vi "_CFX_Sole备份.vi"(0 "CFX cmd":T6, 1 "CFX State":T7, 5 "CFX-config":T2={"neme"="上板机", "CFX Handle"="Cleaner", "Request IP"="amqp://192.168.1.10:5672", "User"="admin", "password"="123456", "Broker IP"="192.168.1.20", "Broker Port"="5672", "Publish Path"="/exchange/Cleaner", "SubPubish Path"="/queue/Broadcast-Cleaner", "Broadcast \nPublish Path"="/exchange/CFX.Host", "Broadcast Sub\npublish Path"="/queue/Broadcast-CFX.Host", "Target \nHandle lD"="CFX.Host", "target IP"="amqp://127.0.0.1", "unit verification"=TRUE, "heartbeat"=FALSE, "timeout period"=5.0}, 7 "CfxData":T1={"Vendor"="YXD", "UniqueIdentifier"="UID5620001", "FriendlyName"="SBJ", "ModelNumber"="SBJ_0001", "SerialNumber"="563210", "NumberofLanes"="2", "CodeIn"="", "CodeOut"="", "Unitldentifer"="", "PositionNumber"="", "PositionName"="", "OldState"="", "NewState"="", "OldStateDuration"="", "Faultcode"="", "Operatorldentifer"="", "LoginName"="", "RecipeName"="", "Revision"="", "Activate formula"="", "Description"=""}, 11 "Error In":errorcluster caption="错误输入", 12 "send?":bool) -> (6 "MessageCFX_out":string, 8 "CFX_Message_In":T3, 14 "ok?":bool, 15 "Error Out":errorcluster caption="错误输出")   [LabVIEW 2025]
uses:
  CFX_dll/CFX.dll
  ctl/CFX-cmd.ctl
  ctl/CfxTopic-cmd.ctl
  ctl/CFX_data.ctl
  ctl/CFX-config.ctl
  SubVI/table/1 model/a log/_myType runlog cmd.ctl
panel:
  out "QueueName":string
  out "IsOpen":bool
  in  "CFX.Host?":bool
  in  "enable?":bool
  out "TraceMessage_EVE":refnum<k27>
  out "TraceMessage":string
  out "AooLog":refnum<k24>
  out "TestSubscribeChannel":bool
  out "TestPublishChannel":bool
  out "log":string
  out "error out":errorcluster
  out "objAMQP_MSG":refnum<k27>
  out "Connection":T4 {"ConnectionEstablished" items=["ConnectionEstablished", "ConnectionFailed", "ConnectionInterrupted", "ConnectionClosed"]}
  out "objAMQP_Request":refnum<k27>
  out "SubscribeChannel":refnum<k24>
  out "return":T5={"CFXHandle"="Cleaner", "RequestNetworkUri"="amqp://10.33.191.97:5672", "RequestTargetAddress"="/queue/Cleaner", "CFX_Message_In"={"Message_Name"="", "Message_Content"=""}, "CFX_Message_out"={"Message_Name"="", "Message_Content"=""}, "CFX_data"=refnum}
  out "FromListener":string
  in  "EndpointInformation":string
  in  "NewState":i32(ring)=1000 items=["PRD"=1000, "PRD_RegularWork"=1100, "PRD_WorkForThirdParties"=1200, "PRD_Rework"=1300, "PRD_Engineering"=1400, "SBY"=2000, "SBY_NoOperator"=2100, "SBY_NoProduct"=2200, "SBY_NoSupportTool"=2300, "SBY_AssociatedClusterModuleDown"=2400, "SBY_NoHost"=2500, "ENG"=3000, "ENG_ProcessExperiments"=3100, "ENG_EquipmentExperiments"=3200, "SDT"=4000, "SDT_UserMaintenanceDelay"=4100, "SDT_SuppliedMaintenanceDelay"=4200, "SDT_PreventiveMaintenance"=4300, "SDT_ChangeOfConsumables"=4400, "SDT_Setup"=4500, "SDT_ProductionTest"=4600, "SDT_FacilitiesRelated"=4700, "USD"=5000, "USD_UserMaintentanceDelay"=5100, "USD_SuppliedMaintenanceDelay"=5200, "USD_Repair"=5300, "USD_OutOfSpecInputMaterial"=5400, "USD_ChangeOfConsumables"=5500, "USD_FacilitiesRelated"=5600, "NST"=6000, "NST_UnworkedShifts"=6100, "NST_EquipmentInstallation"=6200, "NST_EquipmentModifications"=6300, "NST_OfflineTraining"=6400, "NST_ShutdownAndStartup"=6500]
  in  "Broker Url":string="amqp://admin:123456@10.33.191.54:5672"
  out "PublishChannel":refnum<k24>
  in  "rngNewState":i32(ring) items=["PRD"=1000, "PRD_RegularWork"=1100, "PRD_WorkForThirdParties"=1200, "PRD_Rework"=1300, "PRD_Engineering"=1400, "SBY"=2000, "SBY_NoOperator"=2100, "SBY_NoProduct"=2200, "SBY_NoSupportTool"=2300, "SBY_AssociatedClusterModuleDown"=2400, "SBY_NoHost"=2500, "ENG"=3000, "ENG_ProcessExperiments"=3100, "ENG_EquipmentExperiments"=3200, "SDT"=4000, "SDT_UserMaintenanceDelay"=4100, "SDT_SuppliedMaintenanceDelay"=4200, "SDT_PreventiveMaintenance"=4300, "SDT_ChangeOfConsumables"=4400, "SDT_Setup"=4500, "SDT_ProductionTest"=4600, "SDT_FacilitiesRelated"=4700, "USD"=5000, "USD_UserMaintentanceDelay"=5100, "USD_SuppliedMaintenanceDelay"=5200, "USD_Repair"=5300, "USD_OutOfSpecInputMaterial"=5400, "USD_ChangeOfConsumables"=5500, "USD_FacilitiesRelated"=5600, "NST"=6000, "NST_UnworkedShifts"=6100, "NST_EquipmentInstallation"=6200, "NST_EquipmentModifications"=6300, "NST_OfflineTraining"=6400, "NST_ShutdownAndStartup"=6500]
  # "此端点的唯一 CFX 句柄。"
  # "节点队列名"
  # "amqp://10.33.191.64:5672"
  # "amqp://localhost:5672"
  # "Laser"
  # "amqp://192.168.1.20:5672"
  # "AMQP 源或目标的网络地址。可以包括 user 和 port 信息 标准 Uri 格式。（例如：amqps://user1:password1@myamqpbroker.company1.com、amqp://broker3.company1.com、 amqps://myamqpbroker.company1.com:8856 等）。"
  # "本地消息源\nRequest Source"
  # "代理层\nBroker"
  # "请求目标\nRequest Target"
  # "可配置项"
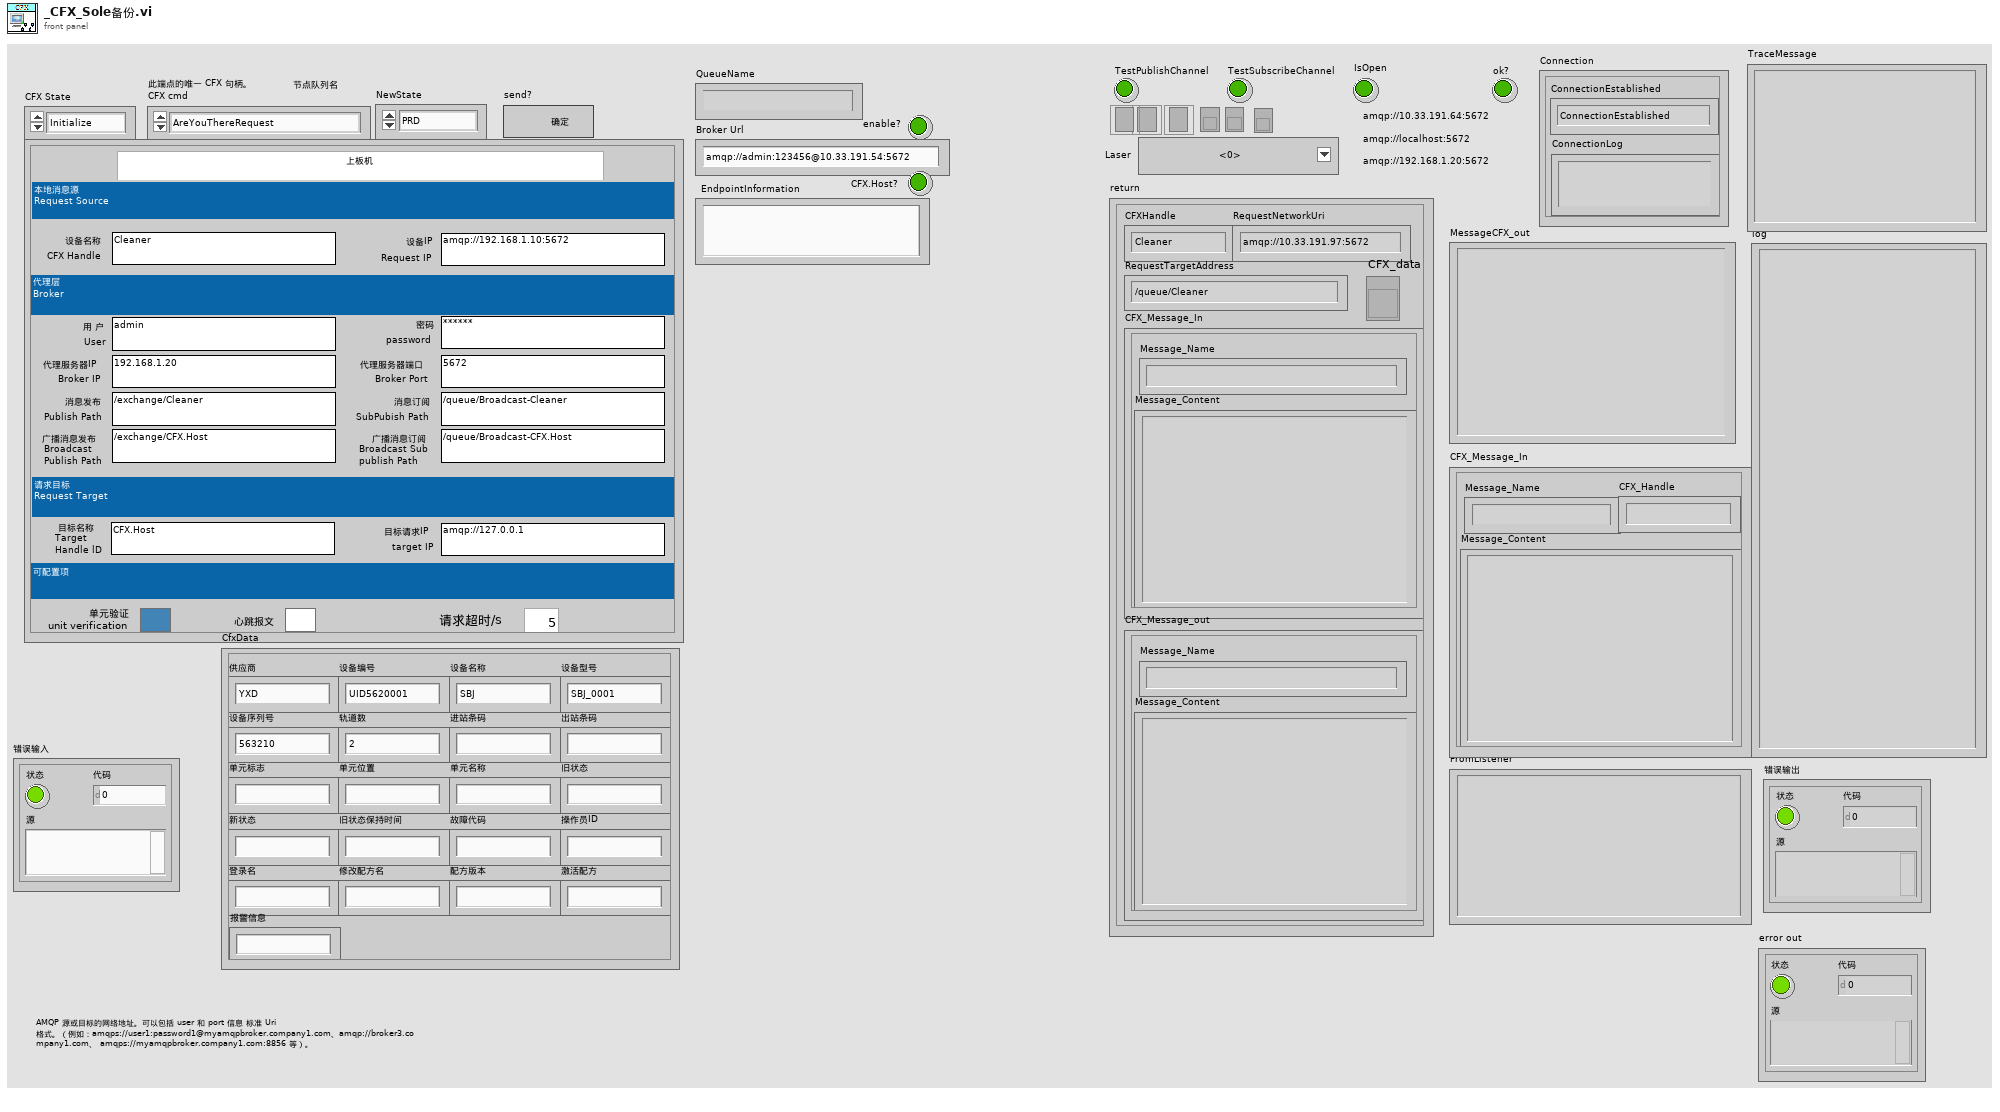
[diagram p1: front panel]
types:
  T1 = typedef "CFX_data.ctl" = cluster{"Vendor":string, "UniqueIdentifier":string, "FriendlyName":string, "ModelNumber":string, "SerialNumber":string, "NumberofLanes":string, "CodeIn":string, "CodeOut":string, "Unitldentifer":string, "PositionNumber":string, "PositionName":string, "OldState":string, "NewState":string, "OldStateDuration":string, "Faultcode":string, "Operatorldentifer":string, "LoginName":string, "RecipeName":string, "Revision":string, "Activate formula":string, "Description":string}
  T2 = typedef "CFX-config.ctl" = cluster{"neme":string, "CFX Handle":string, "Request IP":string, "User":string, "password":string, "Broker IP":string, "Broker Port":string, "Publish Path":string, "SubPubish Path":string, "Broadcast \nPublish Path":string, "Broadcast Sub\npublish Path":string, "Target \nHandle lD":string, "target IP":string, "unit verification":bool, "heartbeat":bool, "timeout period":dbl}
  T3 = cluster{"Message_Name":string, "CFX_Handle":string, "Message_Content":string}
  T4 = cluster{"ConnectionEstablished":i32, "ConnectionLog":string}
  T5 = cluster{"CFXHandle":string, "RequestNetworkUri":string, "RequestTargetAddress":string, "CFX_Message_In":cluster{"Message_Name":string, "Message_Content":string}, "CFX_Message_out":cluster{"Message_Name":string, "Message_Content":string}, "CFX_data":refnum<vi>}
  T6 = typedef "CfxTopic-cmd.ctl" = enum16{"AreYouThereRequest", "AreYouThereResponse", "EndpointConnected", "EndpointShuttingDown", "GetEndpointInformationRequest", "GetEndpointInformationResponse", "Heartbeat", "NotSupportedResponse", "WhoIsThereRequest", "WhoIsThereResponse", "UnitArrived", "UnitsDeparted", "StationStateChanged", "FaultOccurred", "FaultCleared", "OperatorActivated", "OperatorDeactivated", "RecipeModified", "RecipeActived", "ActivateRecipeRequest", "ActivateRecipeResponse"}
  T7 = typedef "CFX-cmd.ctl" = enum16{"Initialize", "Event", "Connection test", "OpenConnection", "Idle", "Shutdown", "WorkComplete", "StationStateChanged", "MaterialsApplied", "CFX", "Hermes"}
  T8 = typedef "_myType runlog cmd.ctl" = enum16{"init", "push (-1: error)", "push (0: user)", "push (1: logical)", "push (2: driver)", "push (3: lib-core)", "push (4: reserved)", "pop", "more?"}
  T9 = cluster{"CFXHandle":string, "RequestNetworkUri":string, "RequestTargetAddress":string, "CFX_Message_In":cluster{"Message_Name":string, "Message_Content":string}, "CFX_Message_out":cluster{"Message_Name":string, "Message_Content":string}, "CFX_data 2":refnum<vi>}
  T10 = typedef "LVStringsAndValuesArrayTypeDef_I32.ctl" = cluster{"String":string, "Value":i32}[]
  T11 = cluster{"Message_Name":string, "Message_Content":string}
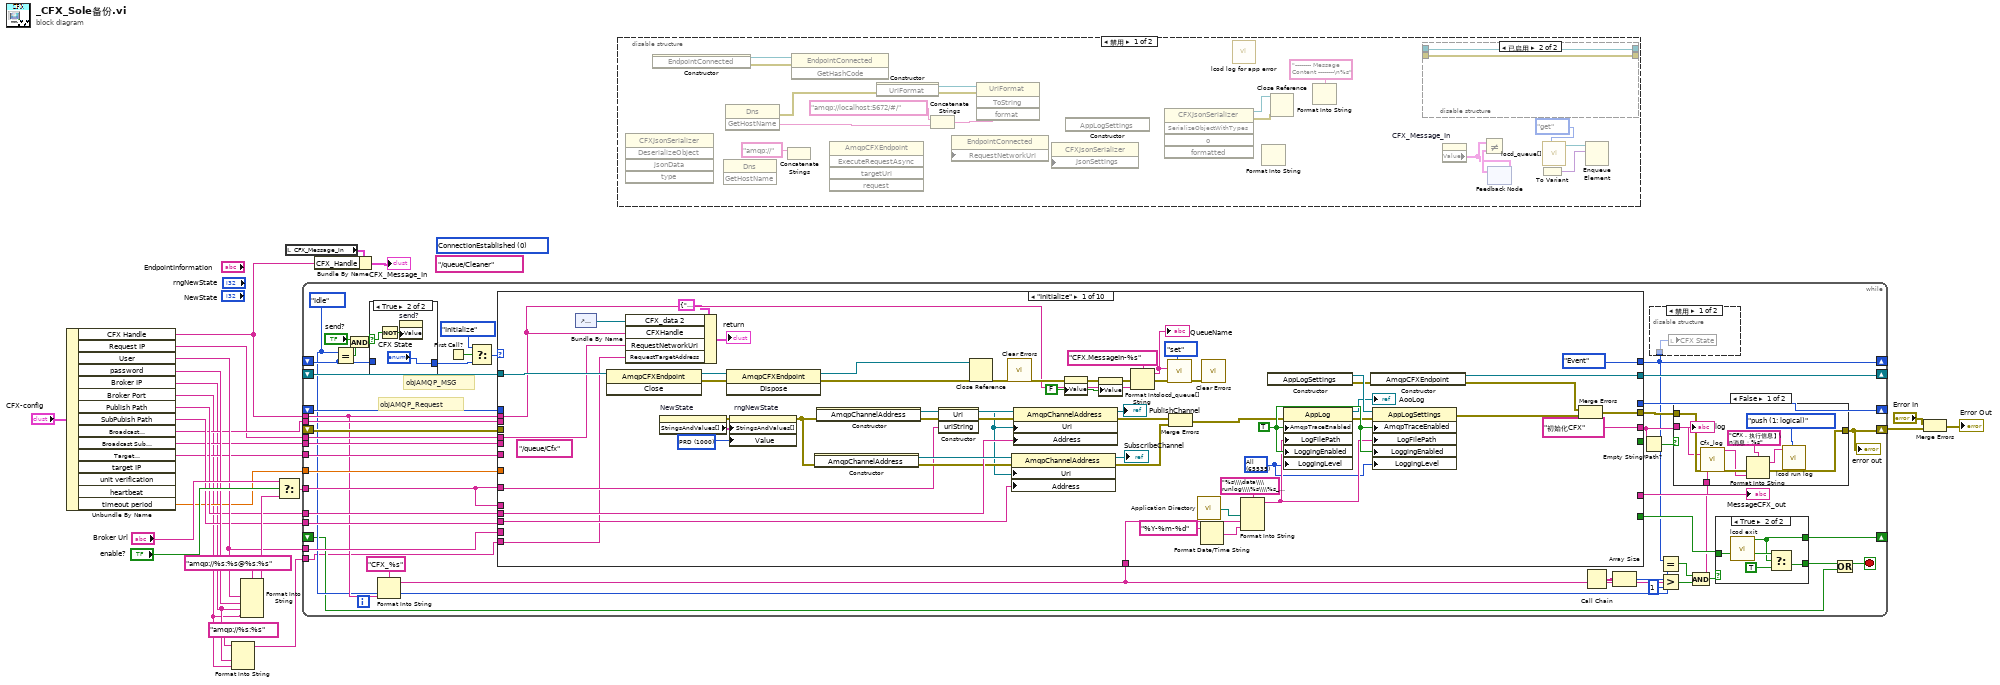
[diagram p0: block diagram]
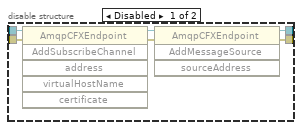
[diagram p2: hidden frame]
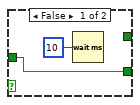
[diagram p6: hidden frame]
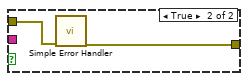
[diagram p7: hidden frame]
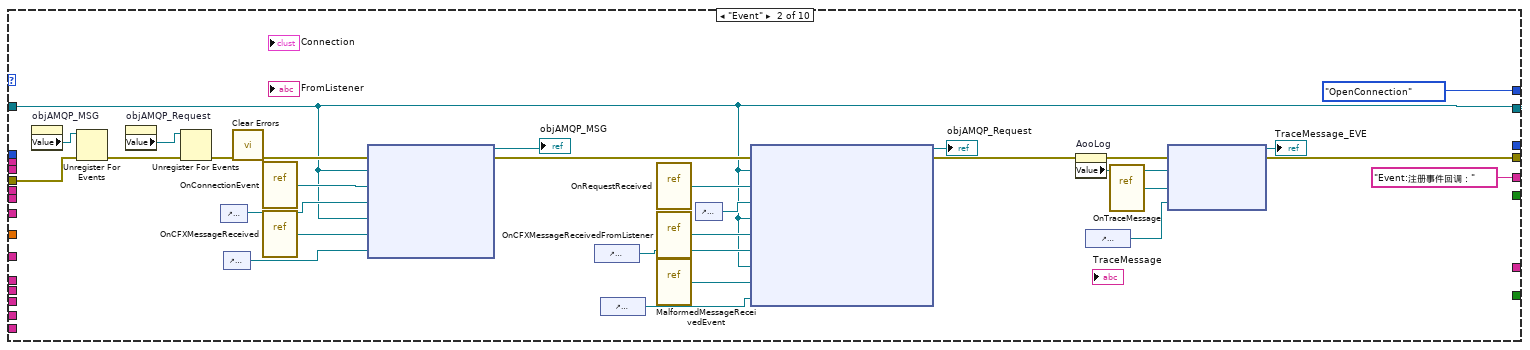
[diagram p8: hidden frame]
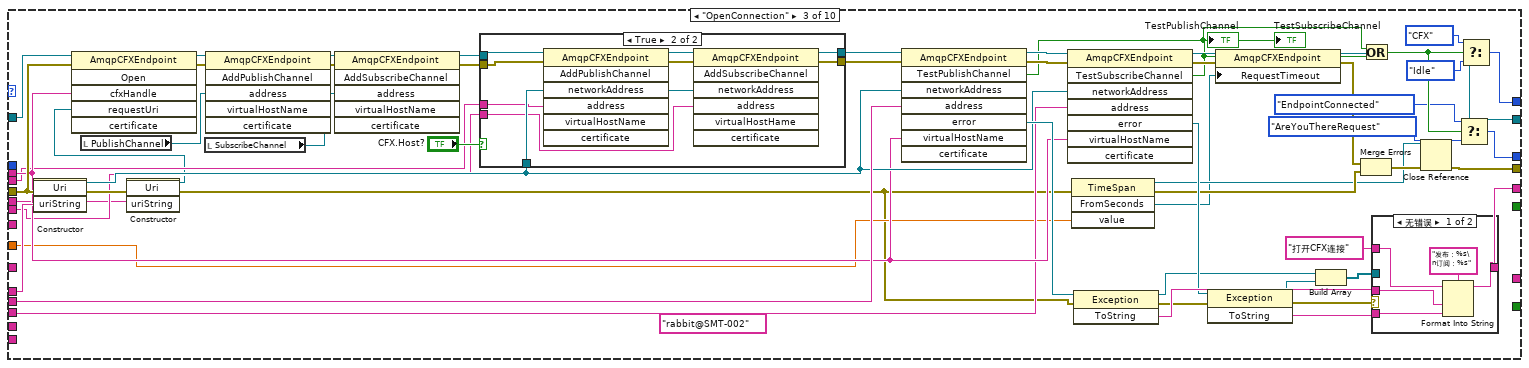
[diagram p9: hidden frame]
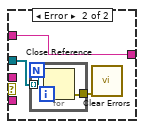
[diagram p11: hidden frame]
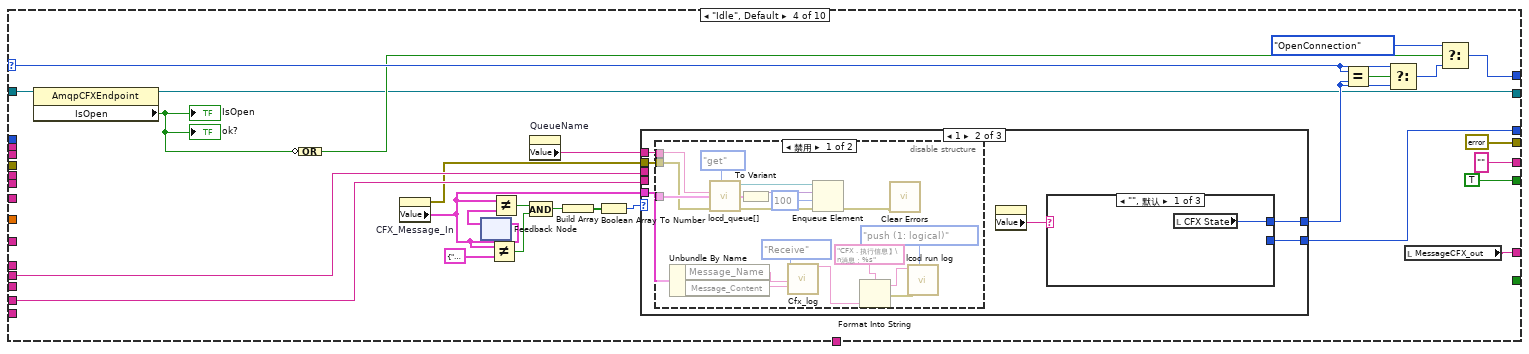
[diagram p12: hidden frame]
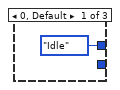
[diagram p13: hidden frame]
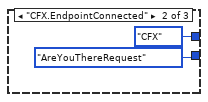
[diagram p15: hidden frame]
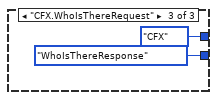
[diagram p16: hidden frame]
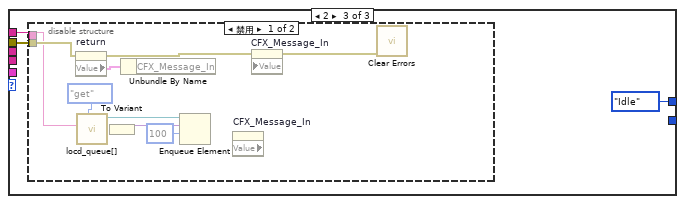
[diagram p17: hidden frame]
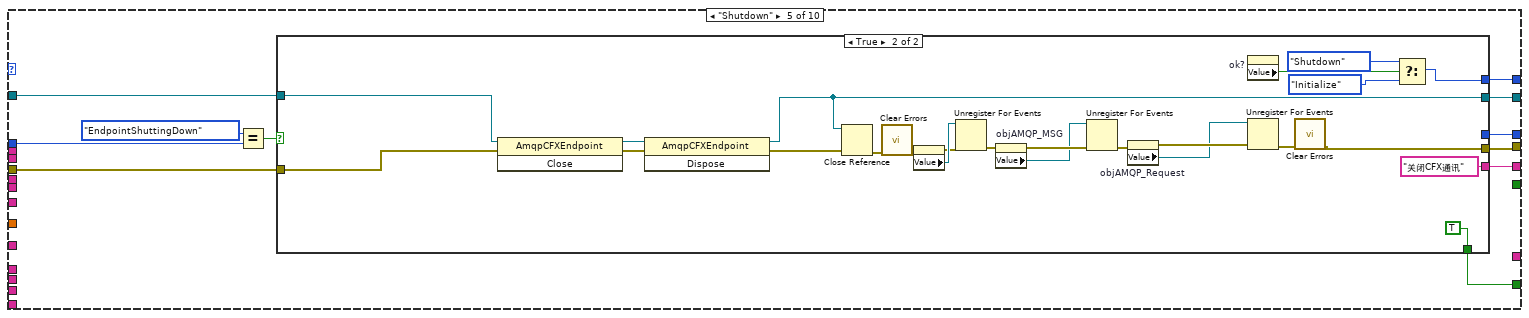
[diagram p19: hidden frame]
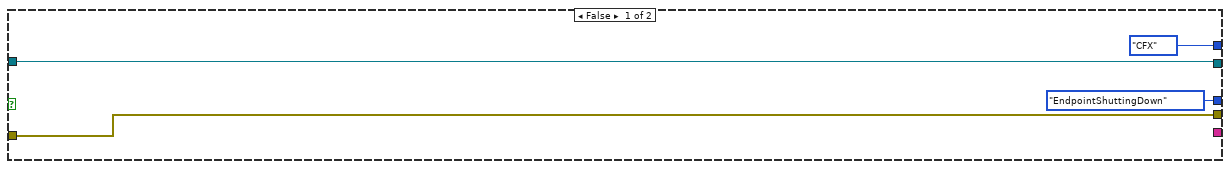
[diagram p20: hidden frame]
diagram:
  (unwired) "/queue/Cleaner" ("RequestTargetAddress")
  (unwired) 0 items=["ConnectionEstablished", "ConnectionFailed", "ConnectionInterrupted", "ConnectionClosed"] ("ConnectionEstablished")
  n1 = Unbundle By Name("CFX-config") -> ("CFX Handle"=w7:string, "Request IP"=w10:string, "User"=w18:string, "password"=w17:string, "Broker IP"=w3:string, "Broker Port"=w2:string, "Publish Path"=w16:string, "SubPubish Path"=w15:string, "Broadcast \nPublish Path"=w14:string, "Broadcast Sub\npublish Path"=w13:string, "Target \nHandle lD"=w12:string, "timeout period"=w11:dbl)  [unwired: 3 out]
  n2 = Format Into String(format string="amqp://%s:%s" ("格式字符串"), w3, w2) -> (resulting string=w1:string)  [unwired: 2 in, 1 out]
  n3 = Format Into String(format string="amqp://%s:%s@%s:%s" ("格式字符串"), w18, w17, w3, w2) -> (resulting string=w20:string)  [unwired: 2 in, 1 out]
  n4 = Select(t="Broker Url", s="enable?", f=w20) -> (s? t:f=w9:string)
  n5 = local read "CFX_Message_In"() -> (w6:T3)
  n6 = while {
    shift-right: [w45] -> _
    shift-left: _ -> [w34]
    shift-right: [w68] -> _
    shift-left: _ -> [w69]
    shift-right: [w62] -> w8
    shift-left: _ -> [w56]
    shift-right: [w61] -> _
    shift-left: _ -> [w63]
    tunnel: w9 -> [w57]
    tunnel: w15 -> [w60]
    tunnel: w16 -> [w59]
    tunnel: w7 -> [w39]
    tunnel: w18 -> [w58]
    tunnel: w10 -> [w55]
    tunnel: w14 -> [w54]
    tunnel: w13 -> [w53]
    tunnel: w12 -> [w52]
    tunnel: w11 -> [w51]
    shift-right: [w35] -> _
    shift-left: _ -> [w29]
    tunnel: w1 -> [w26]
    stop <- w30 stop-if-true
    w33 = CFX-cmd."Idle" ("CFX State")
    # "objAMQP_Request"
    # "objAMQP_MSG"
    n7 = Equal?(x=w33, y=w34) -> (x = y?=w31:bool)
    n8 = And(x="send?", y=w31) -> (x .and. y?=w32:bool)
    n9 = case shown="True" w32 {
      selector: w32 -> [_ w73]
      tunnel: w34 -> [w71 _]
      tunnel: [w71 "CFX State"] -> w38
      frame False {
      }
      frame True {
        n10 = Not(x=w73) -> (.not. x?=w72:bool)
        n11 = property on="send?" class="Bool (严格)"("Value"=w72) -> ()  [unwired: 2 in, 2 out]
      }
    }
    n12 = Format Into String(format string="CFX_%s" ("log_path"), w39) -> (resulting string=w37:string)  [unwired: 2 in, 1 out]
    n13 = First Call?() -> (First Call?: T/F=w27:bool)
    n14 = Select(t=CFX-cmd."Initialize" ("CFX State"), s=w27, f=w38) -> (s? t:f=w41:T7)
    n15 = case shown="\"Initialize\"" w41 {
      selector: w41 -> [_ _ _ w280 _ _ _ _ _ _]
      tunnel: [_ _ _ _ w326 _ _ _ _ _] -> w47
      tunnel: w69 -> [w128 w149 w232 w269 w332 w376 w404 w429 w469 w487]
      tunnel: [w134 w149 w189 w254 w328 w375 w402 w428 w468 w486] -> w68
      tunnel: [w129 w168 w203 errorcluster {"status"=FALSE, "code"=0, "source"=""} ("error out") w327 w372 w399 w427 w479 w485] -> w67
      tunnel: [_ _ _ w279 _ w367 w391 w414 w463 w484] -> w66
      tunnel: [_ _ _ TRUE _ _ _ _ _ _] -> _
      tunnel: ["初始化CFX" ("格式字符串") "Event:注册事件回调：" ("SerializeObjectWithTypes") w225 "" ("SerializeObjectWithTypes") w331 w364 w391 w413 w473 w484] -> w65
      tunnel: [CFX-cmd."Event" ("CFX State") CFX-cmd."OpenConnection" ("CFX State") w196 w264 w330 CFX-cmd."Idle" ("CFX State") CFX-cmd."Idle" ("CFX State") CFX-cmd."Idle" ("CFX State") w449 CFX-cmd."Idle" ("CFX State")] -> w45
      tunnel: w56 -> [_ w163 w206 _ w329 w362 w389 w411 w470 w482]
      tunnel: w63 -> [_ _ _ _ w325 _ _ _ w453 _]
      tunnel: [_ _ w192 w274 w322 _ _ _ w448 _] -> w61
      tunnel: w57 -> [w101 _ _ _ _ _ _ _ _ _]
      tunnel: w60 -> [w119 _ w185 _ _ _ _ _ _ _]
      tunnel: w59 -> [w118 _ w215 w271 _ _ _ _ _ _]
      tunnel: w39 -> [w104 _ w199 _ _ _ _ _ w446 _]
      tunnel: w58 -> [_ _ _ w270 _ _ _ _ _ _]
      tunnel: w57 -> [_ _ w214 _ _ _ _ _ _ _]
      tunnel: w55 -> [w105 _ w183 _ _ _ _ _ _ _]
      tunnel: w54 -> [_ _ w187 _ _ _ _ _ _ _]
      tunnel: w53 -> [_ _ w186 _ _ _ _ _ _ _]
      tunnel: w52 -> [_ _ _ _ _ _ _ _ w445 _]
      tunnel: w51 -> [_ _ w184 _ _ _ _ _ _ _]
      tunnel: w37 -> [w103 _ _ _ _ _ _ _ _ _]
      tunnel: w26 -> [w94 _ _ _ _ _ _ _ _ _]
      frame "Initialize" {
        (unwired) "/queue/Cfx" ("RequestTargetAddress")
        w123 = FALSE ("TestPublishChannel")
        w131 = 65535 items=["Debug"=1, "Info"=2, "Warn"=4, "Error"=8, "All"=65535] ("LoggingLevel")
        w133 = TRUE ("LoggingEnabled")
        w145 = 1000 items=["PRD"=1000, "PRD_RegularWork"=1100, "PRD_WorkForThirdParties"=1200, "PRD_Rework"=1300, "PRD_Engineering"=1400, "SBY"=2000, "SBY_NoOperator"=2100, "SBY_NoProduct"=2200, "SBY_NoSupportTool"=2300, "SBY_AssociatedClusterModuleDown"=2400, "SBY_NoHost"=2500, "ENG"=3000, "ENG_ProcessExperiments"=3100, "ENG_EquipmentExperiments"=3200, "SDT"=4000, "SDT_UserMaintenanceDelay"=4100, "SDT_SuppliedMaintenanceDelay"=4200, "SDT_PreventiveMaintenance"=4300, "SDT_ChangeOfConsumables"=4400, "SDT_Setup"=4500, "SDT_ProductionTest"=4600, "SDT_FacilitiesRelated"=4700, "USD"=5000, "USD_UserMaintentanceDelay"=5100, "USD_SuppliedMaintenanceDelay"=5200, "USD_Repair"=5300, "USD_OutOfSpecInputMaterial"=5400, "USD_ChangeOfConsumables"=5500, "USD_FacilitiesRelated"=5600, "NST"=6000, "NST_UnworkedShifts"=6100, "NST_EquipmentInstallation"=6200, "NST_EquipmentModifications"=6300, "NST_OfflineTraining"=6400, "NST_ShutdownAndStartup"=6500] ("NewState")
        n16 = control-ref of="CfxData"() -> (w93:refnum<vi>)
        n17 = invoke class="AmqpCFXEndpoint" method="Close"(reference=w128) -> (reference out=w126:refnum<k24>, error out=w95:errorcluster)  [unwired: 2 in, 1 out]
        n18 = Bundle By Name(cluster=T9 {"CFXHandle"="Cleaner", "RequestNetworkUri"="amqp://192.168.1.10:5672", "RequestTargetAddress"="/queue/Cleaner", "CFX_Message_In"={"Message_Name"="", "Message_Content"=""}, "CFX_Message_out"={"Message_Name"="", "Message_Content"=""}, "CFX_data 2"=refnum} ("return"), "CFX_data 2"=w93, "CFXHandle"=w104, "RequestNetworkUri"=w105, "RequestTargetAddress"=w94) -> (→"return":T9)
        n19 = property on="NewState" class="Ring (严格)"() -> (error out=w144:errorcluster, "StringsAndValues[]"=w148:T10)  [unwired: 2 in, 1 out]
        n20 = invoke on="调用节点" class="AmqpCFXEndpoint" method="Dispose"(reference=w126, error in=w95) -> (reference out=w97:refnum<k24>, error out=w96:errorcluster)  [unwired: 1 in, 1 out]
        n21 = property on="rngNewState" class="Ring (严格)"(error in=w144, "StringsAndValues[]"=w148, "Value"=w145) -> (error out=w125:errorcluster)  [unwired: 1 in, 1 out]
        n22 = constructor class="AmqpChannelAddress"(error in=w125) -> (reference out=w138:refnum<k24>, error out=w117:errorcluster)  [unwired: 2 in, 1 out]
        n23 = constructor class="AmqpChannelAddress"(error in=w125) -> (reference out=w143:refnum<k24>, error out=w147:errorcluster)  [unwired: 2 in, 1 out]
        n24 = constructor class="Uri"(error in=w147, "uriString"=w101) -> (reference out=w116:refnum<k24>, error out=w146:errorcluster)  [unwired: 2 in, 2 out]
        n25 = Close Reference(reference=w97, error in (no error)=w96) -> (error out=w127:errorcluster)
        n26 = call <vilib>:"Clear Errors.vi"("error in (no error)"=w127) -> ("error out"=w115:errorcluster)  [unwired: 5 in, 1 out]
        n27 = property class="AmqpChannelAddress"(reference=w138, error in=w117, "Uri"=w116, "Address"=w119) -> (reference out=→"SubscribeChannel":refnum<k24>, error out=w136:errorcluster)
        n28 = property class="AmqpChannelAddress"(reference=w143, error in=w146, "Uri"=w116, "Address"=w118) -> (reference out=→"PublishChannel":refnum<k24>, error out=w137:errorcluster)
        n29 = property on="TestPublishChannel" class="Bool (严格)"(error in=w115, "Value"=w123) -> (error out=w124:errorcluster)  [unwired: 1 in, 1 out]
        n30 = property on="TestSubscribeChannel" class="Bool (严格)"(error in=w124, "Value"=w123) -> (error out=w100:errorcluster)  [unwired: 1 in, 1 out]
        n31 = Format Into String(format string="CFX.MessageIn-%s" ("格式字符串"), error in=w100, w104) -> (resulting string=w109:string, error out=w106:errorcluster)  [unwired: 1 in]
        "QueueName" <- w109
        n32 = call "locd_queue[].vi"("cmd"=enum16{"init", "get", "set", "end"}."set", "error in"=w106, "queue_name"=w109) -> ("error out"=w107:errorcluster)  [unwired: 4 in, 4 out]
        n33 = Merge Errors(w137, w136) -> (w108:errorcluster)
        n34 = call <vilib>:"Application Directory.vi"() -> ("Application Directory"=w142:path)
        n35 = Format Date/Time String(time format string (%c)="%Y-%m-%d" ("格式字符串")) -> (date/time string=w102:string)  [unwired: 2 in]
        n36 = call <vilib>:"Clear Errors.vi"("error in (no error)"=w107) -> ()  [unwired: 5 in, 2 out]
        n37 = Format Into String(format string="%s\\\\data\\\\runlog\\\\%s\\\\%s_cfxDebig.txt" ("格式字符串"), w142, w103, w102) -> (resulting string=w132:string)  [unwired: 2 in, 1 out]
        n38 = constructor class="AppLogSettings"() -> (reference out=w130:refnum<k24>, error out=w122:errorcluster)  [unwired: 3 in, 1 out]
        n39 = property class="AppLog"(error in=w108, "AmqpTraceEnabled"=w133, "LogFilePath"=w132, "LoggingEnabled"=w133, "LoggingLevel"=w131) -> (reference out=→"AooLog":refnum<k24>, error out=w120:errorcluster)  [unwired: 1 in]
        n40 = constructor class="AmqpCFXEndpoint"(error in=w122) -> (reference out=w134:refnum<k24>, error out=w98:errorcluster)  [unwired: 2 in, 1 out]
        n41 = property class="AppLogSettings"(reference=w130, error in=w120, "AmqpTraceEnabled"=w133, "LogFilePath"=w132, "LoggingEnabled"=w133, "LoggingLevel"=w131) -> (error out=w112:errorcluster)  [unwired: 1 out]
        n42 = Merge Errors(w98, w112) -> (w129:errorcluster)
      }
      frame "Event" {
        n43 = property on="objAMQP_MSG" class="Ref (严格)"() -> ("Value"=w152:refnum<k27>)  [unwired: 2 in, 2 out]
        n44 = Unregister For Events(event registration refnum=w152, error in=w163) -> (error out=w153:errorcluster)
        n45 = property on="objAMQP_Request" class="Ref (严格)"() -> ("Value"=w150:refnum<k27>)  [unwired: 2 in, 2 out]
        n46 = Unregister For Events(event registration refnum=w150, error in=w153) -> (error out=w151:errorcluster)
        n47 = control-ref of="Connection"() -> (w175:refnum<vi>)
        n48 = control-ref of="CFX_Message_In"() -> (w160:refnum<vi>)
        n49 = call <vilib>:"Clear Errors.vi"("error in (no error)"=w151) -> ("error out"=w154:errorcluster)  [unwired: 5 in, 1 out]
        n50 = vi-ref "OnConnectionEvent.vi"() -> ("vi reference"=w176:refnum<vi>)
        n51 = vi-ref "OnCFXMessageReceived.vi"() -> ("vi reference"=w161:refnum<vi>)
        n52 = node(w154, w149, w176, w175, w149, w161, w160) -> (→"objAMQP_MSG":refnum<k27>, w159:errorcluster)  [unwired: 1 in]
        n53 = control-ref of="FromListener"() -> (w157:refnum<vi>)
        n54 = control-ref of="FromListener"() -> (w155:refnum<vi>)
        n55 = vi-ref "OnRequestReceived.vi"() -> ("vi reference"=w174:refnum<vi>)
        n56 = vi-ref "OnCFXMessageReceivedFromListener.vi"() -> ("vi reference"=w158:refnum<vi>)
        n57 = vi-ref "MalformedMessageReceivedEvent.vi"() -> ("vi reference"=w156:refnum<vi>)
        n58 = control-ref of="return"() -> (w165:refnum<vi>)
        n59 = node(w159, w149, w174, w165, w149, w158, w157, w149, w156, w155) -> (→"objAMQP_Request":refnum<k27>, w162:errorcluster)  [unwired: 1 in]
        n60 = property on="AooLog" class="Ref (严格)"(error in=w162) -> (error out=w164:errorcluster, "Value"=w170:refnum<k24>)  [unwired: 1 in, 1 out]
        n61 = control-ref of="TraceMessage"() -> (w166:refnum<vi>)
        n62 = vi-ref "OnTraceMessage.vi"() -> ("vi reference"=w169:refnum<vi>)
        n63 = node(w164, w170, w169, w166) -> (→"TraceMessage_EVE":refnum<k27>, w168:errorcluster)  [unwired: 1 in]
      }
      frame "OpenConnection" {
        (unwired) "rabbit@SMT-002" ("sourceAddress")
        n64 = constructor class="Uri"(error in=w206, "uriString"=w214) -> (reference out=w213:refnum<k24>, error out=w211:errorcluster)  [unwired: 2 in, 2 out]
        n65 = local read "PublishChannel"() -> (w227:refnum<k24>)
        n66 = constructor class="Uri"(error in=w211, "uriString"=w183) -> (reference out=w179:refnum<k24>, error out=w178:errorcluster)  [unwired: 2 in, 2 out]
        n67 = invoke class="AmqpCFXEndpoint" method="Open"(reference=w232, error in=w206, "cfxHandle"=w199, "requestUri"=w179) -> (reference out=w210:refnum<k24>, error out=w209:errorcluster)  [unwired: 2 in, 4 out]
        n68 = local read "SubscribeChannel"() -> (w228:refnum<k24>)
        n69 = invoke class="AmqpCFXEndpoint" method="AddPublishChannel"(reference=w210, error in=w209, "address"=w227) -> (reference out=w231:refnum<k24>, error out=w230:errorcluster)  [unwired: 3 in, 4 out]
        n70 = invoke class="AmqpCFXEndpoint" method="AddSubscribeChannel"(reference=w231, error in=w230, "address"=w228) -> (reference out=w207:refnum<k24>, error out=w200:errorcluster)  [unwired: 3 in, 4 out]
        n71 = case shown="True" "CFX.Host?" {
          tunnel: w213 -> [_ w243]
          tunnel: [w233 w242] -> w212
          tunnel: [w234 w241] -> w208
          tunnel: w207 -> [w234 w240]
          tunnel: w200 -> [w233 w237]
          tunnel: w187 -> [_ w236]
          tunnel: w186 -> [_ w235]
          frame False {
          }
          frame True {
            n72 = invoke class="AmqpCFXEndpoint" method="AddPublishChannel"(reference=w240, error in=w237, "networkAddress"=w243, "address"=w236) -> (reference out=w238:refnum<k24>, error out=w239:errorcluster)  [unwired: 3 in, 5 out]
            n73 = invoke class="AmqpCFXEndpoint" method="AddSubscribeChannel"(reference=w238, error in=w239, "networkAddress"=w243, "address"=w235) -> (reference out=w241:refnum<k24>, error out=w242:errorcluster)  [unwired: 3 in, 5 out]
          }
        }
        n74 = invoke on="调用节点" class="AmqpCFXEndpoint" method="TestPublishChannel"(reference=w208, error in=w212, "networkAddress"=w213, "address"=w215, "virtualHostName"=w199) -> (reference out=w226:refnum<k24>, error out=w217:errorcluster, "TestPublishChannel"=w198:bool, "error"=w223:refnum<k24>)  [unwired: 3 in, 4 out]
        "TestPublishChannel" <- w198
        n75 = invoke on="调用节点" class="AmqpCFXEndpoint" method="TestSubscribeChannel"(reference=w226, error in=w217, "networkAddress"=w213, "address"=w185, "virtualHostName"=w199) -> (reference out=w224:refnum<k24>, error out=w205:errorcluster, "TestSubscribeChannel"=w197:bool, "error"=w220:refnum<k24>)  [unwired: 3 in, 4 out]
        "TestSubscribeChannel" <- w197
        n76 = invoke class="TimeSpan" method="FromSeconds"(error in=w178, "value"=w184) -> (reference out=w202:refnum<k24>, error out=w204:errorcluster, "FromSeconds"=w188:refnum<k24>)  [unwired: 2 in, 1 out]
        n77 = invoke class="Exception" method="ToString"(reference=w223, error in=w178) -> (reference out=w182:refnum<k24>, error out=w221:errorcluster, "ToString"=w222:string)  [unwired: 1 in]
        n78 = invoke class="Exception" method="ToString"(reference=w220, error in=w221) -> (reference out=w181:refnum<k24>, error out=w218:errorcluster, "ToString"=w219:string)  [unwired: 1 in]
        n79 = property on="属性节点" class="AmqpCFXEndpoint"(reference=w224, "RequestTimeout"=w188) -> (reference out=w189:refnum<k24>)  [unwired: 1 in, 1 out]
        n80 = Build Array(w182, w181) -> (w180:refnum<k24>[])
        n81 = Merge Errors(w205, w204) -> (w216:errorcluster)
        n82 = Or(x=w198, y=w197) -> (x .or. y?=w193:bool)
        n83 = case shown="无错误" w218 {
          tunnel: "打开CFX连接" ("格式字符串") -> [w248 w251]
          tunnel: [w247 w251] -> w225
          tunnel: w222 -> [w245 _]
          tunnel: w219 -> [w244 _]
          tunnel: w180 -> [_ w250]
          frame No Error {
            n84 = Format Into String(format string="发布：%s\n订阅：%s" ("格式字符串"), initial string=w248, w245, w244) -> (resulting string=w247:string)  [unwired: 1 in, 1 out]
          }
          frame Error {
            n85 = for {
              tunnel: w250 -> [w253] mode=indexing
              tunnel: [w252] -> w249
              n86 = Close Reference(reference=w253) -> (error out=w252:errorcluster)  [unwired: 1 in]
            }
            n87 = call <vilib>:"Clear Errors.vi"("error in (no error)"=w249) -> ()  [unwired: 5 in, 2 out]
          }
        }
        n88 = Close Reference(reference=w202, error in (no error)=w216) -> (error out=w203:errorcluster)
        n89 = Select(t=CfxTopic-cmd."EndpointConnected" ("CFX cmd"), s=w193, f=CfxTopic-cmd."AreYouThereRequest") -> (s? t:f=w192:T6)
        n90 = Select(t=CFX-cmd."CFX" ("CFX State"), s=w193, f=CFX-cmd."Idle" ("CFX State")) -> (s? t:f=w196:T7)
      }
      frame "Idle", Default {
        n91 = property on="属性节点" class="AmqpCFXEndpoint"(reference=w269) -> (reference out=w254:refnum<k24>, "IsOpen"=w268:bool)  [unwired: 1 in, 1 out]
        "IsOpen" <- w268
        "ok?" <- w268
        n92 = Compound Arithmetic op=OR ("复合运算")(invert w268) -> (w255:bool)
        n93 = property on="CFX_Message_In" class="Clust (严格)"() -> (error out=w267:errorcluster, "Value"=w259:T3)  [unwired: 2 in, 1 out]
        n94 = feedback-in #1(w259) -> ()
        n95 = feedback #1() -> (w272:T3)  [unwired: 1 in]
        n96 = Not Equal?(x=w259, y=T3 {"Message_Name"="", "CFX_Handle"="", "Message_Content"=""} ("CFX_Message_In")) -> (x != y?=w257:bool)
        n97 = Not Equal?(x=w259, y=w272) -> (x != y?=w263:bool)
        n98 = And(x=w263, y=w257) -> (x .and. y?=w258:bool)
        n99 = property on="QueueName" class="Str"() -> ("Value"=w260:string)  [unwired: 2 in, 2 out]
        n100 = Build Array(w258) -> (w261:bool[])
        n101 = Boolean Array To Number(Boolean array=w261) -> (number=w262:u32)
        n102 = case shown="1" w262 {
          tunnel: [_ w287 _] -> w274
          tunnel: [CFX-cmd."Idle" ("CFX State") w286 CFX-cmd."Idle" ("CFX State")] -> w273
          tunnel: w271 -> [_ _ _]
          tunnel: w270 -> [_ _ _]
          tunnel: w259 -> [_ w284 _]
          tunnel: w267 -> [_ w282 w312]
          tunnel: w260 -> [_ w283 w310]
          frame 0, Default {
          }
          frame 1 {
            n103 = disable-structure shown="禁用" {
              disable-tunnel: w284 -> [w300 _]
              disable-tunnel: w283 -> [w290 _]
              disable-tunnel: w282 -> [w289 _]
              frame Disabled {
                n104 = Unbundle By Name(w300) -> ("Message_Name"=w299:string, "Message_Content"=w298:string)
                n105 = call "locd_queue[].vi"("cmd"=enum16{"init", "get", "set", "end"}."get", "error in"=w289, "queue_name"=w290) -> ("error out"=w301:errorcluster, "queue_out"=w303:refnum<queue>)  [unwired: 4 in, 3 out]
                n106 = To Variant(anything=w300) -> (Variant=w302:variant)
                n107 = call "Cfx_log.vi"("R/W"=enum16{"Send", "Receive"}."Receive", "Message_Name"=w299, "Message_Content"=w298) -> ("Log_out"=w292:string)  [unwired: 15 in, 1 out]
                n108 = Enqueue Element(queue=w303, element=w302, timeout in ms (-1)=100 ("超时毫秒(-1)"), error in (no error)=w301) -> (error out=w288:errorcluster)  [unwired: 2 out]
                n109 = Format Into String(format string="CFX . 执行信息】\n消息：%s", w292) -> (resulting string=w295:string, error out=w296:errorcluster)  [unwired: 2 in]
                n110 = call <vilib>:"Clear Errors.vi"("error in (no error)"=w288) -> ()  [unwired: 5 in, 2 out]
                n111 = call "lcod run log.vi"("cmd"=_myType_runlog_cmd."push (1: logical)", "Error In"=w296, "str in"=w295) -> ()  [unwired: 6 in, 3 out]
              }
              frame Enabled {
              }
            }
            n112 = property on="Message_Name" class="Str"() -> ("Value"=w285:string)  [unwired: 2 in, 2 out]
            n113 = case shown="\"\", 默认" w285 {
              tunnel: [_ CfxTopic-cmd."AreYouThereRequest" ("CFX cmd") CfxTopic-cmd."WhoIsThereResponse" ("CFX cmd")] -> w287
              tunnel: [w305 CFX-cmd."CFX" ("CFX State") CFX-cmd."CFX" ("CFX State")] -> w286
              frame "", Default {
                n114 = local read "CFX State"() -> (w305:T7)
              }
              frame "CFX.EndpointConnected" {
              }
              frame "CFX.WhoIsThereRequest" {
              }
            }
          }
          frame 2 {
            n115 = disable-structure shown="禁用" {
              disable-tunnel: w312 -> [w318 _]
              disable-tunnel: w310 -> [w313 _]
              frame Disabled {
                n116 = property on="return" class="Clust (严格)"(error in=w318) -> (error out=w320:errorcluster, "Value"=w319:T5)  [unwired: 1 in, 1 out]
                n117 = call "locd_queue[].vi"("cmd"=enum16{"init", "get", "set", "end"}."get", "queue_name"=w313) -> ("queue_out"=w317:refnum<queue>)  [unwired: 5 in, 4 out]
                n118 = To Variant() -> (Variant=w316:variant)  [unwired: 1 in]
                n119 = Unbundle By Name(w319) -> ()  [unwired: 1 out]
                n120 = Enqueue Element(queue=w317, element=w316, timeout in ms (-1)=100 ("超时毫秒(-1)")) -> ()  [unwired: 1 in, 3 out]
                n121 = property on="CFX_Message_In" class="Clust (严格)" props=["Value"]() -> ()  [unwired: 2 in, 3 out]
                n122 = property on="CFX_Message_In" class="Clust (严格)" props=["Value"](error in=w320) -> (error out=w321:errorcluster)  [unwired: 2 in, 1 out]
                n123 = call <vilib>:"Clear Errors.vi"("error in (no error)"=w321) -> ()  [unwired: 5 in, 2 out]
              }
              frame Enabled {
              }
            }
          }
        }
        n124 = Equal?(x=w280, y=w273) -> (x = y?=w275:bool)
        n125 = Select(t=w280, s=w275, f=w273) -> (s? t:f=w265:T7)
        n126 = local read "MessageCFX_out"() -> (w279:string)
        n127 = Select(t=CFX-cmd."OpenConnection" ("CFX State"), s=w255, f=w265) -> (s? t:f=w264:T7)
      }
      frame "Shutdown" {
        n128 = Equal?(x=CfxTopic-cmd."EndpointShuttingDown" ("CFX cmd"), y=w325) -> (x = y?=w323:bool)
        n129 = case shown="True" w323 {
          tunnel: w332 -> [w335 w342]
          tunnel: [_ "关闭CFX通讯" ("格式字符串")] -> w331
          tunnel: [CFX-cmd."CFX" ("CFX State") w339] -> w330
          tunnel: w329 -> [w334 w358]
          tunnel: [w335 w341] -> w328
          tunnel: [w334 w340] -> w327
          tunnel: [_ TRUE] -> w326
          tunnel: [CfxTopic-cmd."EndpointShuttingDown" ("CFX cmd") _] -> w322
          frame False {
          }
          frame True {
            n130 = invoke on="调用节点" class="AmqpCFXEndpoint" method="Close"(reference=w342, error in=w358) -> (reference out=w356:refnum<k24>, error out=w357:errorcluster)  [unwired: 1 in, 1 out]
            n131 = invoke on="调用节点" class="AmqpCFXEndpoint" method="Dispose"(reference=w356, error in=w357) -> (reference out=w341:refnum<k24>, error out=w355:errorcluster)  [unwired: 1 in, 1 out]
            n132 = Close Reference(reference=w341, error in (no error)=w355) -> (error out=w350:errorcluster)
            n133 = call <vilib>:"Clear Errors.vi"("error in (no error)"=w350) -> ("error out"=w349:errorcluster)  [unwired: 5 in, 1 out]
            n134 = property on="TraceMessage_EVE" class="Ref (严格)"(error in=w349) -> (error out=w353:errorcluster, "Value"=w354:refnum<k27>)  [unwired: 1 in, 1 out]
            n135 = Unregister For Events(event registration refnum=w354, error in=w353) -> (error out=w348:errorcluster)
            n136 = property on="objAMQP_MSG" class="Ref (严格)"(error in=w348) -> (error out=w347:errorcluster, "Value"=w346:refnum<k27>)  [unwired: 1 in, 1 out]
            n137 = Unregister For Events(event registration refnum=w346, error in=w347) -> (error out=w345:errorcluster)
            n138 = property on="objAMQP_Request" class="Ref (严格)"(error in=w345) -> (error out=w344:errorcluster, "Value"=w343:refnum<k27>)  [unwired: 1 in, 1 out]
            n139 = property on="ok?" class="Bool (严格)"() -> ("Value"=w338:bool)  [unwired: 2 in, 2 out]
            n140 = Unregister For Events(event registration refnum=w343, error in=w344) -> (error out=w352:errorcluster)
            n141 = call <vilib>:"Clear Errors.vi"("error in (no error)"=w352) -> ("error out"=w340:errorcluster)  [unwired: 5 in, 1 out]
            n142 = Select(t=CFX-cmd."Shutdown" ("CFX State"), s=w338, f=CFX-cmd."Initialize") -> (s? t:f=w339:T7)
          }
        }
      }
      frame "WorkComplete" {
        w384 = 0 items=["Completed", "Failed", ""] ("Result")
        n143 = constructor class="WorkStarted"(error in=w362) -> (reference out=w385:refnum<k24>, error out=w382:errorcluster)  [unwired: 2 in, 1 out]
        n144 = property class="WorkStarted"(reference=w385, error in=w382) -> (error out=w381:errorcluster, "TransactionID"=w383:refnum<k24>)  [unwired: 1 out]
        n145 = constructor class="WorkCompleted"(error in=w381) -> (reference out=w380:refnum<k24>, error out=w379:errorcluster)  [unwired: 2 in, 1 out]
        n146 = property class="WorkCompleted"(reference=w380, error in=w379, "Result"=w384, "TransactionID"=w383) -> (reference out=w370:refnum<k24>, error out=w378:errorcluster)
        n147 = constructor class="CFXEnvelope"() -> (reference out=w387:refnum<k24>, error out=w386:errorcluster)  [unwired: 3 in, 1 out]
        n148 = property class="CFXEnvelope"(reference=w387, error in=w386, "MessageBody"=w370) -> (reference out=w373:refnum<k24>, error out=w374:errorcluster, "MessageName"=w368:string)
        n149 = invoke class="AmqpCFXEndpoint" method="Publish"(reference=w376, error in=w378, "env"=w373) -> (reference out=w375:refnum<k24>, error out=w377:errorcluster)  [unwired: 1 in, 2 out]
        n150 = invoke on="调用节点" class="CFXJsonSerializer" method="SerializeObjectWithTypes"("o"=w370, "formatted"=TRUE) -> (reference out=w369:refnum<k24>, error out=w371:errorcluster, "SerializeObjectWithTypes"=w367:string)  [unwired: 3 in, 2 out]
        n151 = Close Reference(reference=w369, error in (no error)=w371) -> (error out=w365:errorcluster)
        n152 = Merge Errors(w377, w374) -> (w372:errorcluster)
        n153 = Format Into String(format string="\n-------- Message Content --------\n%s" ("格式字符串"), initial string=w368, error in=w365, w367) -> (resulting string=w364:string)  [unwired: 1 out]
      }
      frame "StationStateChanged" {
        n154 = constructor class="StationStateChanged"(error in=w389) -> (reference out=w409:refnum<k24>, error out=w408:errorcluster)  [unwired: 2 in, 1 out]
        n155 = local read "rngNewState"() -> (w403:i32)
        n156 = property class="StationStateChanged"(reference=w409, error in=w408, "NewState"=w403) -> (reference out=w395:refnum<k24>, error out=w405:errorcluster)
        n157 = constructor class="CFXEnvelope"() -> (reference out=w406:refnum<k24>, error out=w407:errorcluster)  [unwired: 3 in, 1 out]
        n158 = property class="CFXEnvelope"(reference=w406, error in=w407, "MessageBody"=w395) -> (reference out=w398:refnum<k24>, error out=w400:errorcluster, "MessageName"=w393:string)
        n159 = invoke class="AmqpCFXEndpoint" method="Publish"(reference=w404, error in=w405, "env"=w398) -> (reference out=w402:refnum<k24>, error out=w401:errorcluster)  [unwired: 1 in, 2 out]
        n160 = invoke on="调用节点" class="CFXJsonSerializer" method="SerializeObjectWithTypes"("o"=w395, "formatted"=TRUE) -> (reference out=w397:refnum<k24>, error out=w396:errorcluster, "SerializeObjectWithTypes"=w391:string)  [unwired: 3 in, 2 out]
        n161 = Close Reference(reference=w397, error in (no error)=w396) -> (error out=w392:errorcluster)
        n162 = Merge Errors(w401, w400) -> (w399:errorcluster)
        n163 = Format Into String(format string="\n-------- Message Content --------%s" ("格式字符串"), initial string=w393, error in=w392, w391) -> ()  [unwired: 2 out]
      }
      frame "MaterialsApplied" {
        n164 = constructor class="MaterialsApplied"(error in=w411) -> (reference out=w434:refnum<k24>, error out=w436:errorcluster)  [unwired: 2 in, 1 out]
        n165 = constructor class="InstalledMaterial"() -> (reference out=w432:refnum<k24>, error out=w433:errorcluster)  [unwired: 3 in, 1 out]
        n166 = invoke class="Guid" method="NewGuid"(error in=w436) -> (error out=w437:errorcluster, "NewGuid"=w435:refnum<k24>)  [unwired: 2 in, 1 out]
        n167 = property class="MaterialsApplied"(reference=w434, error in=w437, "TransactionId"=w435) -> (reference out=w443:refnum<k24>, error out=w424:errorcluster, "AppliedMaterials"=w438:refnum<k24>)
        n168 = property class="InstalledMaterial"(reference=w432, error in=w433, "QuantityInstalled"=1.0, "QuantityNonInstalled"=2.0) -> (reference out=w439:refnum<k24>, error out=w421:errorcluster)
        n169 = Merge Errors(w424, w421) -> (w422:errorcluster)
        n170 = invoke class="List`1[[CFX.Structures.Installe" method="Add"(reference=w438, error in=w422, "item"=w439) -> (reference out=w440:refnum<k24>, error out=w423:errorcluster)  [unwired: 1 in, 2 out]
        n171 = property class="MaterialsApplied"(reference=w443, error in=w423, "AppliedMaterials"=w440) -> (reference out=w417:refnum<k24>, error out=w425:errorcluster)
        n172 = constructor class="CFXEnvelope"(error in=w425) -> (reference out=w441:refnum<k24>, error out=w442:errorcluster)  [unwired: 2 in, 1 out]
        n173 = property class="CFXEnvelope"(reference=w441, error in=w442, "MessageBody"=w417) -> (reference out=w420:refnum<k24>, error out=w426:errorcluster, "MessageName"=w415:string)
        n174 = invoke class="AmqpCFXEndpoint" method="Publish"(reference=w429, error in=w426, "env"=w420) -> (reference out=w428:refnum<k24>, error out=w427:errorcluster)  [unwired: 1 in, 2 out]
        n175 = invoke on="调用节点" class="CFXJsonSerializer" method="SerializeObjectWithTypes"("o"=w417, "formatted"=TRUE) -> (reference out=w418:refnum<k24>, error out=w419:errorcluster, "SerializeObjectWithTypes"=w414:string)  [unwired: 3 in, 2 out]
        n176 = Close Reference(reference=w418, error in (no error)=w419) -> ()  [unwired: 1 out]
        n177 = Format Into String(format string="\n-------- Message Content --------\n%s" ("格式字符串"), initial string=w415, w414) -> (resulting string=w413:string)  [unwired: 1 in, 1 out]
      }
      frame "CFX" {
        w448 = CfxTopic-cmd."EndpointShuttingDown" ("CFX cmd")
        n178 = First Call?() -> (First Call?: T/F=w458:bool)
        n179 = Not Equal?(x=w453, y=CfxTopic-cmd."AreYouThereRequest" ("CFX cmd")) -> (x != y?=w459:bool)
        n180 = property on="return" class="Clust (严格)"() -> ("Value"=w457:T5)  [unwired: 2 in, 2 out]
        n181 = Equal?(x=w448, y=w453) -> (x = y?=w452:bool)
        n182 = Or(x=w459, y=w458) -> (x .or. y?=w460:bool)
        n183 = Unbundle By Name(w457) -> ("CFXHandle"=w456:string, "RequestNetworkUri"=w455:string, "RequestTargetAddress"=w454:string)
        n184 = case shown="True" w460 {
          tunnel: w453 -> [_ w481]
          tunnel: ["CFX cmd" w481] -> w461
          frame False {
          }
          frame True {
          }
        }
        n185 = property on="EndpointInformation" class="Str"(error in=w470) -> (error out=w475:errorcluster, "Value"=w478:string)  [unwired: 1 in, 1 out]
        n186 = call "_lcod_CFX.vi"("RequestTargetAddress"=w454, "RequestNetworkUri"=w455, "cmd"=w461, "Error In"=w475, "in_str"=w478, "CFXHandle"=w456, "CfxData"="CfxData") -> ("Error Out"=w447:errorcluster, "new reference"=w466:refnum<k24>)  [unwired: 2 in, 1 out]
        n187 = Get Date/Time In Seconds() -> (seconds since 1Jan1904=w471:timestamp)
        n188 = property class="CFXEnvelope" props=["CFXVERSION", "MessageName", "Source", "Target", "TimeStamp"](reference=w466, error in=w447, "Source"=w446, "Target"=w445, "TimeStamp"=w471) -> (reference out=w465:refnum<k24>, error out=w472:errorcluster, "MessageName"=w464:string)  [unwired: 1 out]
        n189 = invoke class="AmqpCFXEndpoint" method="Publish"(reference=w469, error in=w472, "env"=w465) -> (reference out=w468:refnum<k24>, error out=w479:errorcluster)  [unwired: 1 in, 2 out]
        n190 = invoke on="调用节点" class="CFXJsonSerializer" method="SerializeObjectWithTypes"("o"=w465, "formatted"=TRUE) -> (reference out=w476:refnum<k24>, error out=w477:errorcluster, "SerializeObjectWithTypes"=w463:string)  [unwired: 3 in, 2 out]
        n191 = Close Reference(reference=w476, error in (no error)=w477) -> ()  [unwired: 1 out]
        n192 = Format Into String(format string="Direction: Send | %s\n-------- Message Content -------\n%s" ("格式字符串"), w464, w463) -> (resulting string=w473:string)  [unwired: 2 in, 1 out]
        n193 = Select(t=CFX-cmd."Shutdown" ("CFX State"), s=w452, f=CFX-cmd."Idle" ("CFX State")) -> (s? t:f=w449:T7)
      }
      frame "Hermes" {
        n194 = disable-structure shown="禁用" {
          disable-tunnel: w487 -> [w490 w492]
          disable-tunnel: [w489 w492] -> w486
          disable-tunnel: [w488 w491] -> w485
          disable-tunnel: [_ ""] -> w484
          disable-tunnel: w482 -> [_ w491]
          frame Disabled {
            n195 = invoke class="AmqpCFXEndpoint" method="Publish"(reference=w490) -> (reference out=w489:refnum<k24>, error out=w488:errorcluster)  [unwired: 3 in, 2 out]
          }
          frame Enabled {
          }
        }
      }
    }
    "MessageCFX_out" <- w66
    n196 = Call Chain() -> (call chain=w50:string[])
    n197 = Array Size(array=w50) -> (size(s)=w49:i32)
    n198 = Empty String/Path?(string/path=w65) -> (empty?=w64:bool)
    n199 = disable-structure shown="禁用" {
      disable-tunnel: w45 -> [w70 _]
      frame Disabled {
        n200 = local write "CFX State"(w70) -> ()
      }
      frame Enabled {
      }
    }
    n201 = Equal?(x=w45, y=w33) -> (x = y?=w42:bool)
    n202 = Greater?(x=w49, y=1) -> (0:w43:bool)
    n203 = case shown="False" w64 {
      tunnel: w67 -> [w89 w91]
      tunnel: [w88 w90] -> w62
      tunnel: w65 -> [w83 _]
      tunnel: w37 -> [w81 _]
      frame False {
        n204 = call "Cfx_log.vi"("login"=w83, "error in"=w89, "log_path"=w81) -> ("Log_out"=w82:string, "error out"=w88:errorcluster)  [unwired: 15 in]
        n205 = Format Into String(format string="CFX . 执行信息】\n消息：%s", w82) -> (resulting string=w86:string, error out=w87:errorcluster)  [unwired: 2 in]
        n206 = call "lcod run log.vi"("cmd"=_myType_runlog_cmd."push (1: logical)", "Error In"=w87, "str in"=w86) -> ()  [unwired: 6 in, 3 out]
        "log" <- w83
      }
      frame True {
        n207 = call <vilib>:"Simple Error Handler.vi"("error in (no error)"=w91) -> ("error out"=w90:errorcluster)  [unwired: 4 in, 4 out]
      }
    }
    "error out" <- w62
    n208 = Compound Arithmetic op=AND ("复合运算")(w42, w43) -> (w44:bool)
    n209 = case shown="True" w44 {
      tunnel: w47 -> [w76 w78]
      tunnel: [w76 w79] -> w46
      tunnel: [_ w77] -> w35
      frame False {
        n210 = Wait (ms)(milliseconds to wait=u32 10 ("等待时间（毫秒）")) -> ()  [unwired: 1 out]
      }
      frame True {
        n211 = call "lcod exit.vi"() -> ("bExit out"=w77:bool)  [unwired: 11 in]
        n212 = Select(t=w78, s=w77, f=TRUE) -> (s? t:f=w79:bool)
      }
    }
    n213 = Or(x=w46, y=w29) -> (x .or. y?=w30:bool)
  }
  n214 = Bundle By Name(cluster=w6, "CFX_Handle"=w7) -> (→"CFX_Message_In":T3)
  n215 = disable-structure shown="禁用" {
    frame Disabled {
      n216 = invoke on="调用节点" class="CFXJsonSerializer" method="DeserializeObject"() -> ()  [unwired: 5 in, 5 out]
      n217 = constructor class="EndpointConnected"() -> (reference out=w503:refnum<k24>, error out=w504:errorcluster)  [unwired: 3 in, 1 out]
      n218 = invoke class="Dns" method="GetHostName"() -> ()  [unwired: 3 in, 3 out]
      n219 = invoke class="Dns" method="GetHostName"() -> (error out=w508:errorcluster, "GetHostName"=w505:string)  [unwired: 3 in, 1 out]
      n220 = Concatenate Strings("amqp://") -> ()  [unwired: 1 in, 1 out]
      n221 = invoke on="调用节点" class="EndpointConnected" method="GetHashCode"(reference=w503, error in=w504) -> ()  [unwired: 1 in, 3 out]
      n222 = invoke on="调用节点" class="AmqpCFXEndpoint" method="ExecuteRequestAsync"() -> ()  [unwired: 5 in, 5 out]
      n223 = constructor class="UriFormat"(error in=w508) -> (reference out=w510:refnum<k24>, error out=w509:errorcluster)  [unwired: 2 in, 1 out]
      n224 = Concatenate Strings("amqp://localhost:5672/#/" ("format"), w505) -> (w506:string)
      n225 = property class="EndpointConnected" props=["RequestNetworkUri"]() -> ()  [unwired: 3 in, 2 out]
      n226 = invoke class="UriFormat" method="ToString"(reference=w510, error in=w509, "format"=w506) -> ()  [unwired: 1 in, 4 out]
      n227 = property class="CFXJsonSerializer" props=["JsonSettings"]() -> ()  [unwired: 3 in, 2 out]
      n228 = constructor class="AppLogSettings"() -> ()  [unwired: 3 in, 3 out]
      n229 = invoke on="调用节点" class="CFXJsonSerializer" method="SerializeObjectWithTypes"() -> (reference out=w501:refnum<k24>, error out=w502:errorcluster)  [unwired: 5 in, 3 out]
      n230 = call "lcod log for app error.vi"() -> ()  [unwired: 10 in, 2 out]
      n231 = Format Into String() -> ()  [unwired: 4 in, 2 out]
      n232 = Close Reference(reference=w501, error in (no error)=w502) -> ()  [unwired: 1 out]
      n233 = Format Into String(format string="-------- Message Content --------\n%s" ("格式字符串")) -> ()  [unwired: 3 in, 2 out]
      n234 = disable-structure shown="已启用" {
        disable-tunnel: [w516 w518] -> _
        disable-tunnel: [w515 w517] -> _
        disable-tunnel: _ -> [w514 w518]
        disable-tunnel: _ -> [w513 w517]
        frame Disabled {
          n235 = invoke class="AmqpCFXEndpoint" method="AddSubscribeChannel"(reference=w514, error in=w513) -> (reference out=w512:refnum<k24>, error out=w511:errorcluster)  [unwired: 4 in, 4 out]
          n236 = invoke class="AmqpCFXEndpoint" method="AddMessageSource"(reference=w512, error in=w511) -> (reference out=w516:refnum<k24>, error out=w515:errorcluster)  [unwired: 2 in, 2 out]
        }
        frame Enabled {
        }
      }
      n237 = property on="CFX_Message_In" class="Clust (严格)"() -> ("Value"=w496:T11)  [unwired: 2 in, 2 out]
      n238 = feedback #2() -> (w498:T11)  [unwired: 1 in]
      n239 = Not Equal?(x=w496, y=w498) -> ()  [unwired: 1 out]
      n240 = feedback-in #2(w496) -> ()
      n241 = To Variant() -> (Variant=w495:variant)  [unwired: 1 in]
      n242 = call "locd_queue[].vi"("cmd"=enum16{"init", "get", "set", "end"}."get") -> ("queue_out"=w497:refnum<queue>)  [unwired: 6 in, 4 out]
      n243 = Enqueue Element(queue=w497, element=w495) -> ()  [unwired: 2 in, 3 out]
    }
    frame Enabled {
    }
  }
  n244 = Merge Errors("Error In", w8) -> (→"Error Out":errorcluster)
